vi "Get Children Object.vi"(8 "error in":errorcluster, 10 "Element":string, 11 "json class in":refnum<class "json class.lvclass">) -> (0 "error out":errorcluster, 2 "Children Object":refnum<class "json class.lvclass">, 3 "json class out":refnum<class "json class.lvclass">)   [LabVIEW 2021, in "Config Library.lvlib" / "json class.lvclass"]
uses:
  json class.lvclass
  json class.lvclass/json class.ctl
  <vilib>/addons/JSON API/JSON Value/JSON Value.lvclass
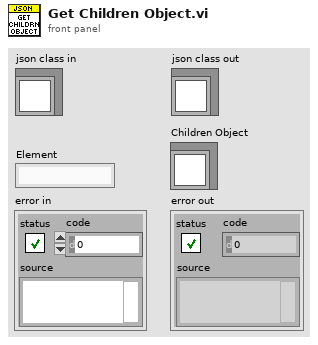
[diagram p1: front panel]
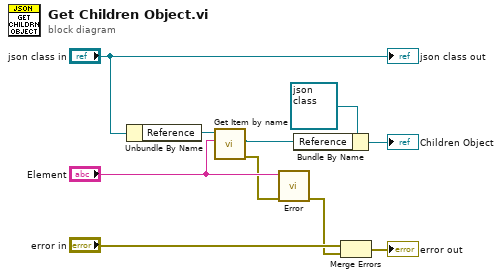
[diagram p0: block diagram]
diagram:
  n1 = Unbundle By Name("json class in") -> ("Reference"=w6:refnum<class "JSON Value.lvclass">)
  n2 = call-dynamic "Get Item by name.vi"("name"="Element", "JSON Value In"=w6) -> ("error out"=w2:errorcluster, "Value"=w5:refnum<class "JSON Value.lvclass">)  [unwired: 6 in, 2 out]
  n3 = call "Error.vi"("error in (no error)"=w2, "Name"="Element") -> ("error out"=w1:errorcluster)  [unwired: 9 in]
  n4 = Bundle By Name(cluster=refnum<class "json class.lvclass"> refnum ("Config Library.lvlib:json class.lvclass"), "Reference"=w5) -> (→"Children Object":refnum<class "json class.lvclass">)
  n5 = Merge Errors("error in", w1) -> (→"error out":errorcluster)
  "json class out" <- "json class in"
